vi "DrawToPictureCore.vi"(5 "Pixel Formats":T1, 7 "Top Left Point":T2, 8 "error in (no error)":errorcluster, 11 "Buffer In":refnum<class "Buffer.lvclass">) -> (0 "error out":errorcluster, 3 "Picture":picture)   [LabVIEW 2020, in "Buffer.lvclass"]
uses:
  Buffer.lvclass
  Picture Top Left Point Offset.ctl
  Pixel Formats.ctl
  Buffer.lvclass/Buffer.ctl
  bin/gindustrialcam_32-1.dll
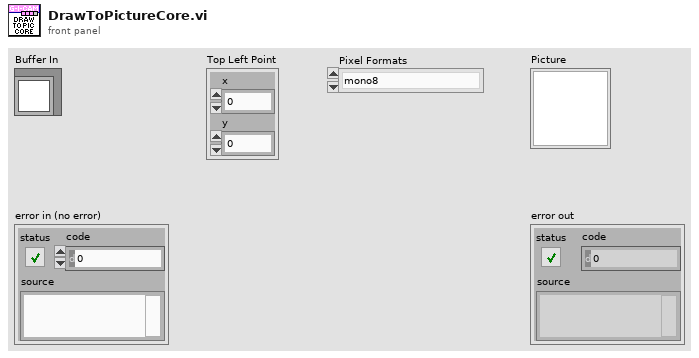
[diagram p1: front panel]
types:
  T1 = typedef "Buffer.lvclass/Pixel Formats.ctl" = enum16{"mono8", "mono10", "mono10p", "mono12", "mono12p", "mono14", "mono14p", "mono16", "RGB8", "BGR8"}
  T2 = typedef "Buffer.lvclass/Picture Top Left Point Offset.ctl" = cluster{"x":i16, "y":i16}
  T3 = cluster{"op_code":i16, "length":i32, "image_bytes_length":i32, "top":i16, "left":i16, "bottom":i16, "right":i16, "bitwidth":i16, "foreground":u32, "background":u32}
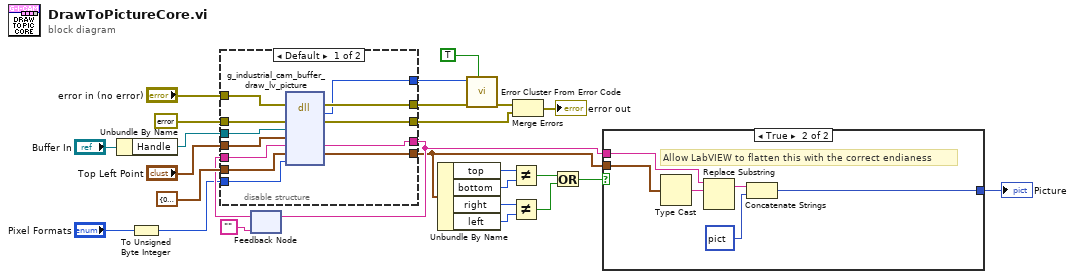
[diagram p0: block diagram]
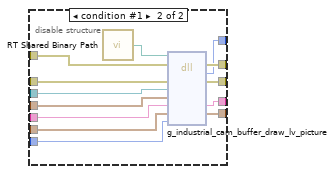
[diagram p2: hidden frame]
diagram:
  n1 = Unbundle By Name("Buffer In") -> ("Handle"=w1:refnum<data-value>)
  n2 = To Unsigned Byte Integer(number="Pixel Formats") -> (unsigned 8bit integer=w2:u8)
  n3 = feedback #1("" ("Empty String Constant")) -> (w14:string)
  n4 = disable-structure shown="Default" {
    disable-tunnel: "Top Left Point" -> [w38 w51]
    disable-tunnel: "error in (no error)" -> [w37 w50]
    disable-tunnel: errorcluster {"status"=FALSE, "code"=0, "source"=""} ("error constant") -> [w36 w49]
    disable-tunnel: T3 {"op_code"=0, "length"=0, "image_bytes_length"=0, "top"=0, "left"=0, "bottom"=0, "right"=0, "bitwidth"=0, "foreground"=0, "background"=0} -> [w35 w48]
    disable-tunnel: [w34 w47] -> w18
    disable-tunnel: [w33 w46] -> w17
    disable-tunnel: [w32 w45] -> w16
    disable-tunnel: [w31 w44] -> w15
    disable-tunnel: w14 -> [w30 w43]
    disable-tunnel: [w29 w42] -> w11
    disable-tunnel: w2 -> [w28 w41]
    disable-tunnel: w1 -> [w27 w40]
    frame condition #0 (active) {
      n5 = dll-call lib="C:/serenial/lib/g-industrial-camera/LabVIEW/g_industrial_cam/bin/gindustrialcam_*-1.*" fn="g_industrial_cam_buffer_draw_lv_picture" ("g_ar_toolkit.*.*:g_ar_tk_image_draw_picture")(error in=w37, "error_cluster"=w36, "EDVR src"=w27, "top_left"=w38, "picture"=w30, "op_header"=w35, "pixel_format"=w28) -> (error out=w34:errorcluster, "return type"=w33:i32, "error_cluster"=w32:errorcluster, "picture"=w31:string, "op_header"=w29:T3)  [unwired: 5 in, 1 out]
    }
    frame condition #1 {
      n6 = call "RT Shared Binary Path.vi"() -> ("Path"=w39:path)
      n7 = dll-call lib="C:/serenial/lib/g-industrial-camera/LabVIEW/g_industrial_cam/bin/gindustrialcam_*-1.*" fn="g_industrial_cam_buffer_draw_lv_picture" ("g_ar_toolkit.*.*:g_ar_tk_image_draw_picture")(path in=w39, error in=w50, "error_cluster"=w49, "EDVR src"=w40, "top_left"=w51, "picture"=w43, "op_header"=w48, "pixel_format"=w41) -> (error out=w47:errorcluster, "return type"=w46:i32, "error_cluster"=w45:errorcluster, "picture"=w44:string, "op_header"=w42:T3)  [unwired: 4 in, 1 out]
    }
  }
  n8 = feedback-in #1(w15) -> ()
  n9 = Unbundle By Name(w11) -> ("top"=w10:i16, "bottom"=w9:i16, "right"=w7:i16, "left"=w6:i16)
  n10 = call <vilib>:"Error Cluster From Error Code.vi"("show call chain? (False)"=TRUE, "error in (no error)"=w18, "error code (0)"=w17) -> ("error out"=w25:errorcluster)  [unwired: 6 in]
  n11 = Not Equal?(x=w10, y=w9) -> (x != y?=w8:bool)
  n12 = Not Equal?(x=w7, y=w6) -> (x != y?=w4:bool)
  n13 = Merge Errors(w25, w16) -> (→"error out":errorcluster)
  n14 = Or(x=w8, y=w4) -> (x .or. y?=w5:bool)
  n15 = case shown="True" w5 {
    tunnel: [_ w55] -> w23
    tunnel: w11 -> [_ w54]
    tunnel: w15 -> [_ w53]
    frame False {
    }
    frame True {
      # "Allow LabVIEW to flatten this with the correct endianess"
      n16 = Type Cast(x=w54) -> (*(type *) &x=w57:string)  [unwired: 1 in]
      n17 = Replace Substring(4:w57, 5:w53) -> (1:w56:string)  [unwired: 2 in, 1 out]
      n18 = Concatenate Strings(w56, picture data[5B] ("empty picture")) -> (w55:picture)
    }
  }
  "Picture" <- w23
